vi "set Swept SA - Marker Auto Search Type.vi"(6 "Auto Search On?":bool, 8 "error in (no error)":errorcluster, 9 "Index":i32, 10 "Marker Auto Type":T1, 11 "Keysight 9020A in":refnum<class "Keysight 9020A.lvclass">) -> (0 "error out":errorcluster, 3 "Keysight 9020A out":refnum<class "Keysight 9020A.lvclass">)   [LabVIEW 2023, in "Spectrum Analyzer.lvlib" / "Keysight 9020A.lvclass"]
uses:
  Keysight 9020A.lvclass
  TYPE DEFINITION/TYPE Marker Auto Select.ctl
  Keysight 9020A.lvclass/Keysight 9020A.ctl
  <vilib>/ErrorRing/Error Ring.xnode
  Spectrum Analyzer.lvlib
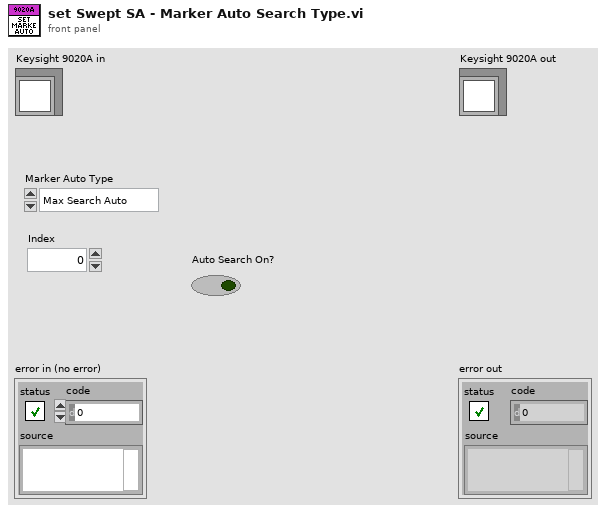
[diagram p1: front panel]
types:
  T1 = typedef "Spectrum Analyzer.lvlib/TYPE Marker Auto Select.ctl" = enum16{"Max Search Auto", "Min Search Auto"}
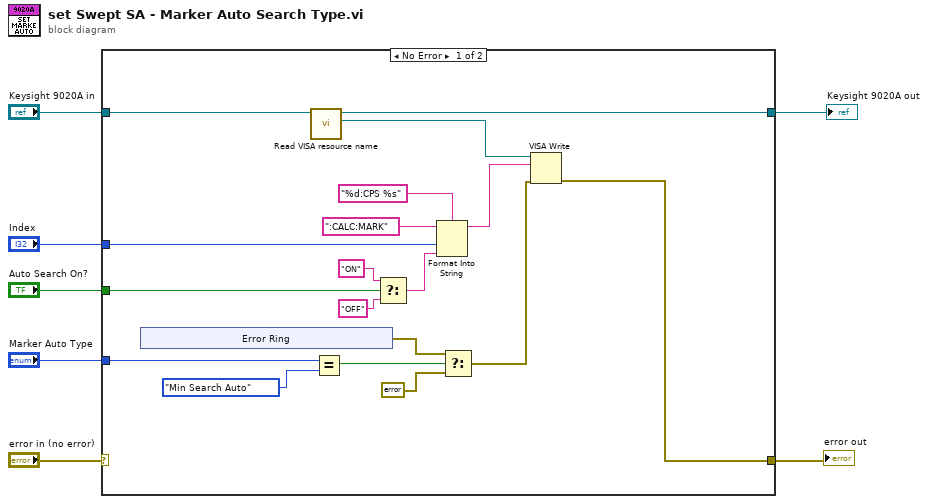
[diagram p0: block diagram]
diagram:
  n1 = case shown="No Error" "error in (no error)" {
    selector: "error in (no error)" -> [_ w27]
    tunnel: "Keysight 9020A in" -> [w25 w28]
    tunnel: [w24 w28] -> w6
    tunnel: [w20 w27] -> w4
    tunnel: "Marker Auto Type" -> [w12 _]
    tunnel: "Index" -> [w16 _]
    tunnel: "Auto Search On?" -> [w8 _]
    frame No Error {
      n2 = xnode "Error Ring"() -> ("error out"=w14:errorcluster)
      n3 = call "Read VISA resource name.vi"("Keysight 9020A in"=w25) -> ("VISA resource name"=w19:refnum<visa-resource-name>, "Keysight 9020A out"=w24:refnum<class "Keysight 9020A.lvclass">)  [unwired: 8 in, 1 out]
      n4 = Equal?(x=w12, y=TYPE_Marker_Auto_Select."Min Search Auto") -> (x = y?=w17:bool)
      n5 = Select(t="ON", s=w8, f="OFF") -> (s? t:f=w9:string)
      n6 = Format Into String(format string="%d:CPS %s", initial string=":CALC:MARK", w16, w9) -> (resulting string=w22:string)  [unwired: 1 in, 1 out]
      n7 = Select(t=w14, s=w17, f=errorcluster {"status"=FALSE, "code"=0, "source"=""}) -> (s? t:f=w15:errorcluster)
      n8 = VISA Write(VISA resource name=w19, write buffer=w22, error in (no error)=w15) -> (error out=w20:errorcluster)  [unwired: 2 out]
    }
    frame Error {
    }
  }
  "error out" <- w4
  "Keysight 9020A out" <- w6
